vi "table_get_subtable_keys.vi"(7 "subtables":string[](array[string]), 8 "error in (no error)":errorcluster, 11 "Table in":refnum<class "Table.lvclass">) -> (0 "error out":errorcluster, 1 "keys":string[](array[string]), 2 "found subtable?":bool, 3 "Table out":refnum<class "Table.lvclass">)   [LabVIEW 2020, in "toml.lvclass"]
uses:
  toml.lvclass
  Table/Table.lvclass
  toml.lvclass/toml.ctl
  Item/Item.lvclass
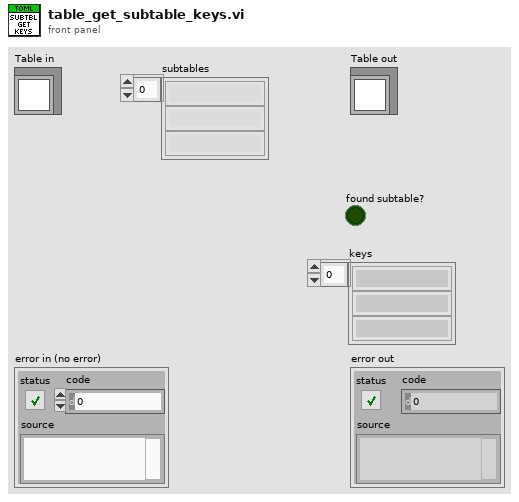
[diagram p1: front panel]
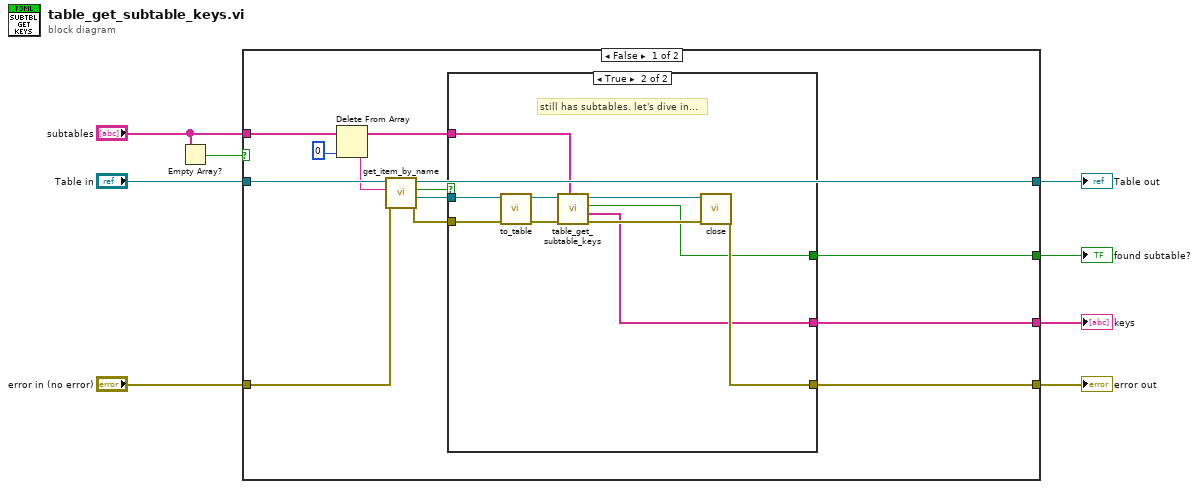
[diagram p0: block diagram]
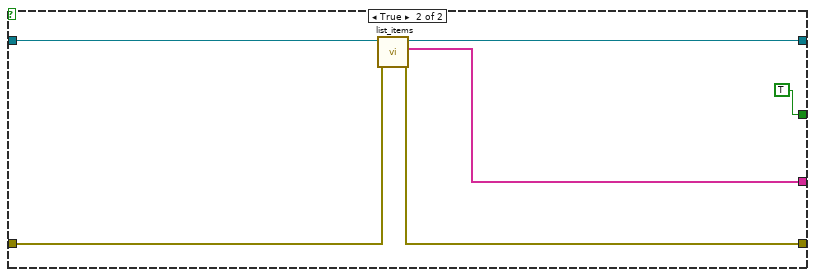
[diagram p3: hidden frame]
diagram:
  n1 = Empty Array?(array="subtables") -> (empty?=w4:bool)
  n2 = case shown="False" w4 {
    tunnel: [w12 w34] -> w8
    tunnel: [w15 w37] -> w7
    tunnel: "Table in" -> [w18 w38]
    tunnel: "error in (no error)" -> [w17 w33]
    tunnel: "subtables" -> [w21 _]
    tunnel: [w11 w36] -> w2
    tunnel: [w10 TRUE ("found subtable?")] -> w1
    frame False {
      n3 = Delete From Array(array=w21, index=0) -> (deleted portion=w13:string, array with subset deleted=w19:string[])  [unwired: 1 in]
      n4 = call "get_item_by_name.vi"("error in (no error)"=w17, "item_name"=w13, "Table in"=w18) -> ("error out"=w14:errorcluster, "Item"=w16:refnum<class "Item.lvclass">, "found?"=w9:bool, "Table out"=w15:refnum<class "Table.lvclass">)  [unwired: 4 in, 1 out]
      n5 = case shown="True" w9 {
        tunnel: w19 -> [_ w32]
        tunnel: w16 -> [_ w31]
        tunnel: w14 -> [w22 w30]
        tunnel: [w22 w27] -> w12
        tunnel: [_ w26] -> w11
        tunnel: [_ w23] -> w10
        frame False {
        }
        frame True {
          # "still has subtables. let's dive in..."
          n6 = call "to_table.vi"("error in (no error)"=w30, "Item in"=w31) -> ("error out"=w25:errorcluster, "Table"=w24:refnum<class "Table.lvclass">)  [unwired: 8 in]
          n7 = call "table_get_subtable_keys.vi"("subtables"=w32, "error in (no error)"=w25, "Table in"=w24) -> ("error out"=w28:errorcluster, "keys"=w26:string[], "found subtable?"=w23:bool, "Table out"=w29:refnum<class "Table.lvclass">)  [unwired: 5 in]
          n8 = call "close.vi"("error in (no error)"=w28, "Table in"=w29) -> ("error out"=w27:errorcluster)  [unwired: 9 in]
        }
      }
    }
    frame True {
      n9 = call "list_items.vi"("error in (no error)"=w33, "Table in"=w38) -> ("error out"=w34:errorcluster, "items"=w36:string[], "Table out"=w37:refnum<class "Table.lvclass">)  [unwired: 7 in]
    }
  }
  "error out" <- w8
  "keys" <- w2
  "Table out" <- w7
  "found subtable?" <- w1
